vi "W14_FailRate.vi"() -> ()   [LabVIEW 2026]
doc: "Use this template to build a VI to use as a subVI."
panel:
  in  "stop":bool
  out "notify engineer":bool
  out "boards in window":i32
  out "FAIL rate %":dbl
  in  "FAIL (this board)":bool
  # "One loop = one board (every 0.1 s). Hold FAIL for 1 s = 10 FAIL boards."
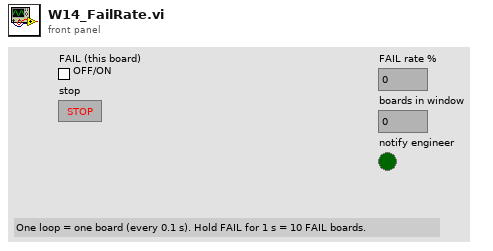
[diagram p1: front panel]
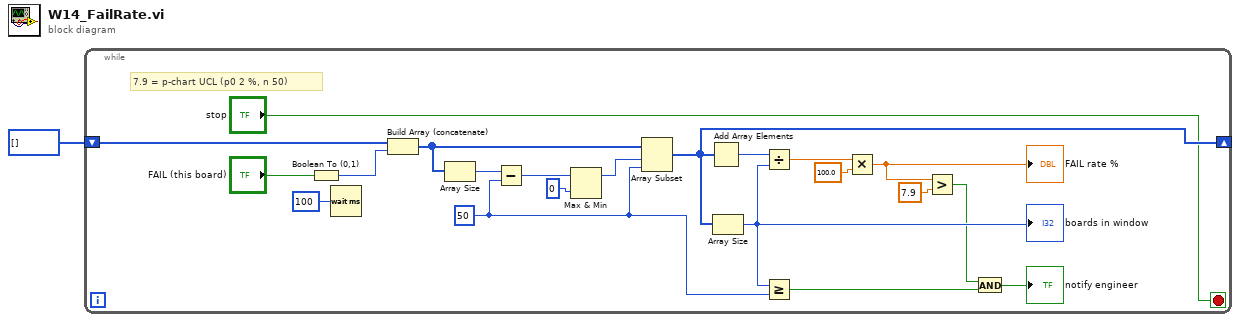
[diagram p0: block diagram]
diagram:
  n1 = while {
    shift-right: [w13] -> _
    shift-left: i16[] [] -> [w21]
    stop <- "stop" stop-if-true
    w17 = 50 ("y")
    # "7.9 = p-chart UCL (p0 2 %, n 50)"
    n2 = Boolean To (0,1)(Boolean="FAIL (this board)") -> (0, 1=w20:i16)
    n3 = Wait (ms)(milliseconds to wait=u32 100) -> ()  [unwired: 1 out]
    n4 = Build Array (concatenate)(w21, w20) -> (w19:i16[])
    n5 = Array Size(array=w19) -> (size(s)=w18:i32)
    n6 = Subtract(x=w18, y=w17) -> (x-y=w16:i32)
    n7 = Max & Min(x=w16, y=0) -> (max(x,y)=w14:i32)  [unwired: 1 out]
    n8 = Array Subset(array=w19, index=w14, length=w17) -> (w13:i16[])
    n9 = Add Array Elements(numeric array=w13) -> (sum=w12:i16)
    n10 = Array Size(array=w13) -> (size(s)=w11:i32)
    "boards in window" <- w11
    n11 = Divide(x=w12, y=w11) -> (x/y=w10:dbl)
    n12 = Greater Or Equal?(x=w11, y=w17) -> (x >= y?=w5:bool)
    n13 = Multiply(x=w10, y=100.0) -> (x*y=w8:dbl)
    "FAIL rate %" <- w8
    n14 = Greater?(x=w8, y=7.9) -> (0:w6:bool)
    n15 = And(x=w6, y=w5) -> (x .and. y?=→"notify engineer":bool)
  }
